vi "S_WriteAttribute.vi"(0 "reference in":refnum<class "SubTemplate.lvclass">, 5 "Error In":errorcluster) -> (14 "reference out":refnum<class "SubTemplate.lvclass">, 19 "Error Out":errorcluster)   [LabVIEW 2020]
uses:
  SubTemplate.lvclass
  BaseTemplate/protected/ObjectAttributes.ctl
  BaseTemplate/BaseTemplate.lvclass
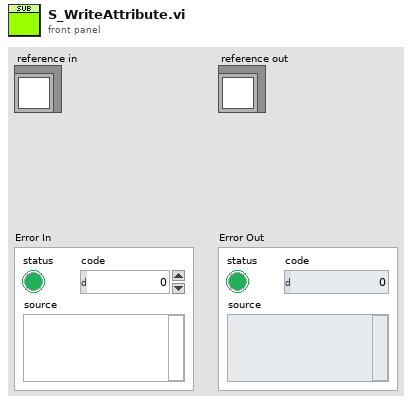
[diagram p1: front panel]
types:
  T1 = typedef "BaseTemplate.lvclass/ObjectAttributes.ctl" = cluster{"Attribute1":dbl}
  T2 = typedef "SubTemplate.lvclass/ObjectAttributes.ctl" = cluster{"Base class":T1}
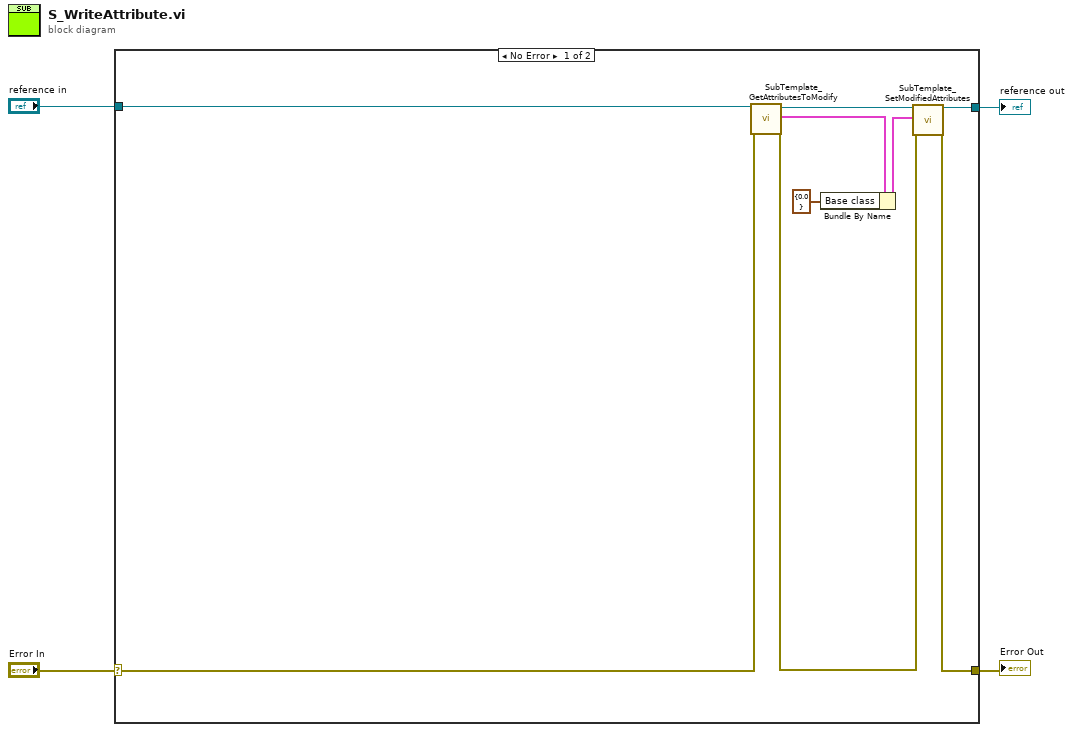
[diagram p0: block diagram]
diagram:
  n1 = case shown="No Error" "Error In" {
    selector: "Error In" -> [w8 w15]
    tunnel: [w10 w15] -> w3
    tunnel: [w7 w14] -> w1
    tunnel: "reference in" -> [w9 w14]
    frame No Error {
      n2 = call "SubTemplate_GetAttributesToModify.vi"("reference in"=w9, "error in (no error)"=w8) -> ("reference out"=w11:refnum<class "SubTemplate.lvclass">, "Attributes"=w13:T2, "error out"=w6:errorcluster)  [unwired: 14 in, 1 out]
      n3 = Bundle By Name(cluster=w13, "Base class"=T1 {"Attribute1"=0.0}) -> (w12:T2)
      n4 = call "SubTemplate_SetModifiedAttributes.vi"("reference in"=w11, "Attributes"=w12, "error in (no error)"=w6) -> ("reference out"=w7:refnum<class "SubTemplate.lvclass">, "error out"=w10:errorcluster)  [unwired: 15 in]
    }
    frame Error {
    }
  }
  "Error Out" <- w3
  "reference out" <- w1
